vi "Launch server.vi"(10 "Lancer server.py":string=" \"D:\\Home\\eschaub\\Documents\\INFORMATIQUE\\LabVIEW-Python TCP\\lancer_serveur.py\"", 11 "Port":u16=5000) -> (3 "Port out":u16=5000)   [LabVIEW 2020, in "LabVIEW-Python TCP Lib.lvlib"]
uses:
  LabVIEW-Python TCP Lib.lvlib
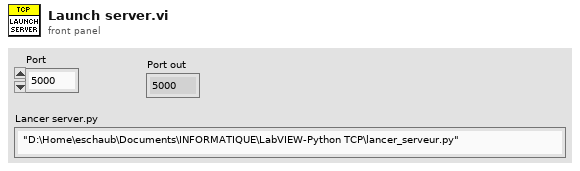
[diagram p1: front panel]
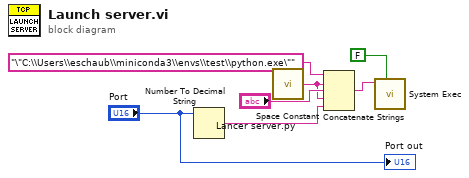
[diagram p0: block diagram]
diagram:
  n1 = Number To Decimal String(number="Port") -> (decimal integer string=w2:string)  [unwired: 1 in]
  n2 = call <vilib>:"Space Constant.vi"() -> ("String"=w3:string)
  n3 = Concatenate Strings("\"C:\\Users\\eschaub\\miniconda3\\envs\\test\\python.exe\"" ("command line"), w3, "Lancer server.py", w3, w2) -> (w4:string)
  n4 = call <vilib>:"System Exec.vi"("wait until completion? (T)"=FALSE, "command line"=w4) -> ()  [unwired: 6 in, 4 out]
  "Port out" <- "Port"
